vi "Map Path.vi"(8 "error in (no error)":errorcluster, 11 "file or folder path pattern":string) -> (0 "error out":errorcluster, 3 "Path Out":path)   [LabVIEW 2021]
doc: "This VI search for a file or folder name and return the fist found full path."
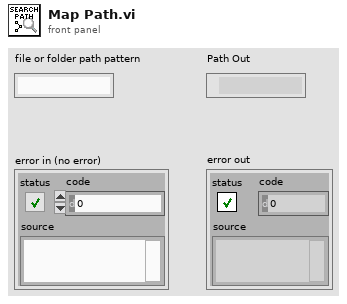
[diagram p1: front panel]
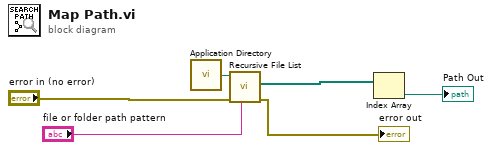
[diagram p0: block diagram]
diagram:
  n1 = call <vilib>:"Application Directory.vi"() -> ("Application Directory"=w1:path)
  n2 = call <vilib>:"Recursive File List.vi"("pattern"="file or folder path pattern", "error in (no error)"="error in (no error)", "Folder Path"=w1) -> ("error out"=→"error out":errorcluster, "All Files in Dir"=w3:path[])  [unwired: 4 in, 3 out]
  n3 = Index Array(array=w3) -> (element=→"Path Out":path)  [unwired: 1 in]
